vi "query Swept SA - Trace Value by CSV file.vi"(8 "error in (no error)":errorcluster, 10 "Trace Index":u32, 11 "Keysight 9020A in":refnum<class "Keysight 9020A.lvclass">) -> (0 "error out":errorcluster, 2 "Trace Values":T1 {"Frequency" format="%#_6p"}, 3 "Keysight 9020A out":refnum<class "Keysight 9020A.lvclass">)   [LabVIEW 2023, in "Spectrum Analyzer.lvlib" / "Keysight 9020A.lvclass"]
uses:
  Keysight 9020A.lvclass
  TYPE DEFINITION/TYPE Trace Value Array.ctl
  Keysight 9020A.lvclass/Keysight 9020A.ctl
  Spectrum Analyzer.lvlib
  <vilib>/Utility/file.llb/Read Delimited Spreadsheet (string).vi
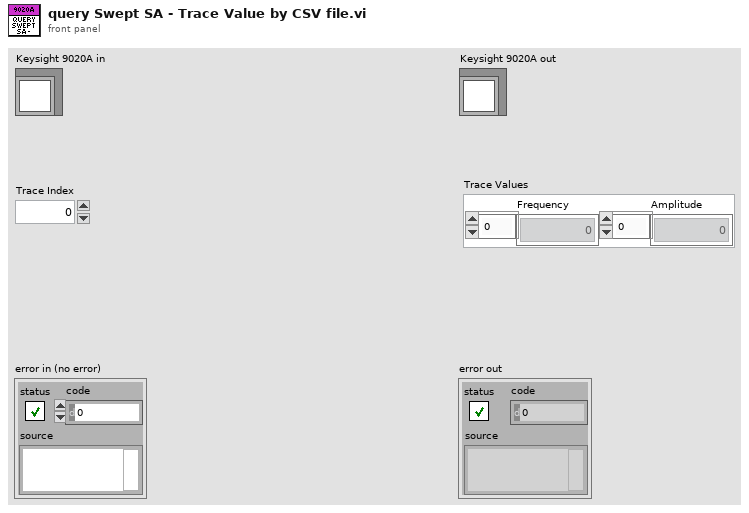
[diagram p1: front panel]
types:
  T1 = typedef "Spectrum Analyzer.lvlib/TYPE Trace Value Array.ctl" = cluster{"Frequency":dbl[], "Amplitude":dbl[]}
  T2 = enum16{"big-endian, network order", "native, host order", "little-endian"}
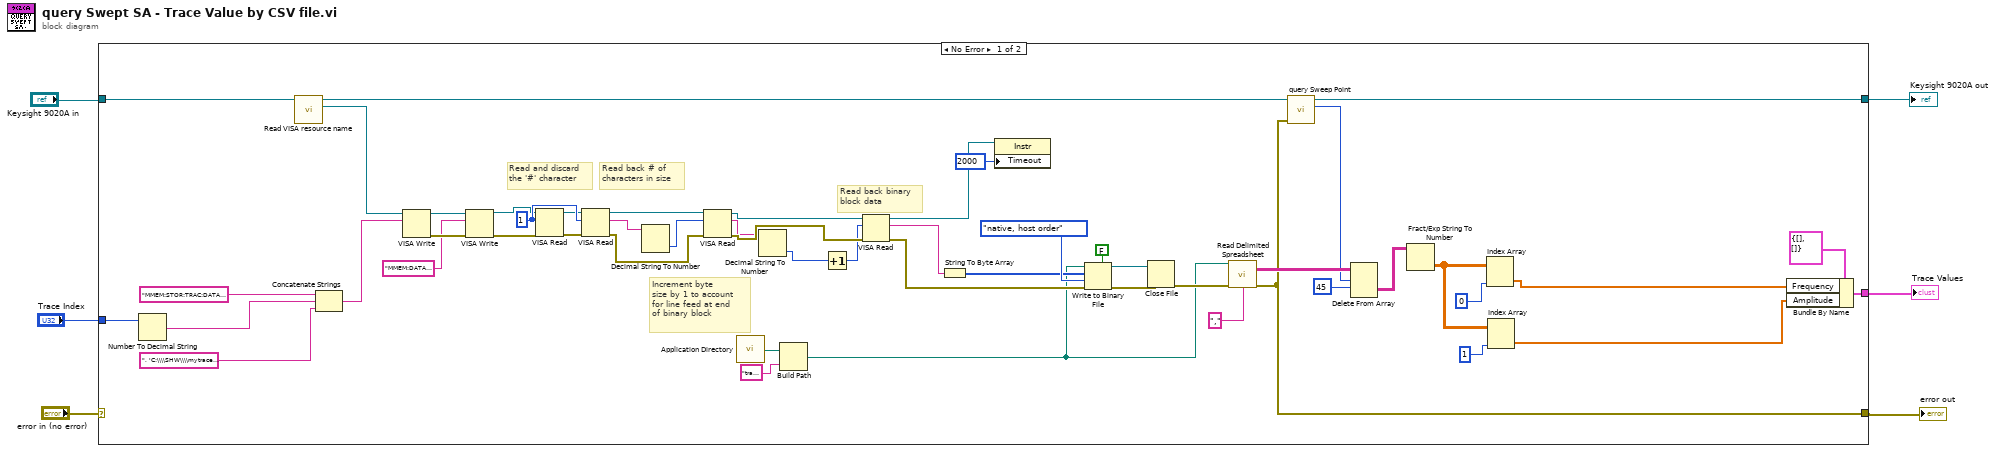
[diagram p0: block diagram]
diagram:
  n1 = case shown="No Error" "error in (no error)" {
    selector: "error in (no error)" -> [_ w59]
    tunnel: "Keysight 9020A in" -> [w58 w60]
    tunnel: [w15 w60] -> w5
    tunnel: [w14 w59] -> w2
    tunnel: "Trace Index" -> [w52 _]
    tunnel: [w56 _] -> w4
    frame No Error {
      w47 = u32 1 ("byte count")
      # "Read back binary\nblock data"
      # "Increment byte\nsize by 1 to account\nfor line feed at end\nof binary block"
      # "Read back # of\ncharacters in size"
      # "Read and discard\nthe '#' character"
      n2 = Number To Decimal String(number=w52) -> (decimal integer string=w54:string)  [unwired: 1 in]
      n3 = call "Read VISA resource name.vi"("Keysight 9020A in"=w58) -> ("VISA resource name"=w12:refnum<visa-resource-name>, "Keysight 9020A out"=w20:refnum<class "Keysight 9020A.lvclass">)  [unwired: 8 in, 1 out]
      n4 = Concatenate Strings("MMEM:STOR:TRAC:DATA TRACE" ("write buffer"), w54, ", 'C:\\\\SHW\\\\mytrace.csv';*OPC" ("write buffer")) -> (w51:string)
      n5 = VISA Write(VISA resource name=w12, write buffer=w51) -> (VISA resource name out=w50:refnum<visa-resource-name>, error out=w49:errorcluster)  [unwired: 1 in, 1 out]
      n6 = VISA Write(VISA resource name=w50, write buffer="MMEM:DATA? 'C:\\\\SHW\\\\mytrace.csv'", error in (no error)=w49) -> (VISA resource name out=w45:refnum<visa-resource-name>, error out=w44:errorcluster)  [unwired: 1 out]
      n7 = VISA Read(VISA resource name=w45, byte count=w47, error in (no error)=w44) -> (VISA resource name out=w46:refnum<visa-resource-name>, error out=w43:errorcluster)  [unwired: 2 out]
      n8 = VISA Read(VISA resource name=w46, byte count=w47, error in (no error)=w43) -> (VISA resource name out=w27:refnum<visa-resource-name>, read buffer=w25:string, error out=w26:errorcluster)  [unwired: 1 out]
      n9 = Decimal String To Number(string=w25) -> (number=w38:i32)  [unwired: 2 in, 1 out]
      n10 = VISA Read(VISA resource name=w27, byte count=w38, error in (no error)=w26) -> (VISA resource name out=w39:refnum<visa-resource-name>, read buffer=w40:string, error out=w42:errorcluster)  [unwired: 1 out]
      n11 = call <vilib>:"Application Directory.vi"() -> ("Application Directory"=w24:path)
      n12 = Decimal String To Number(string=w40) -> (number=w41:i32)  [unwired: 2 in, 1 out]
      n13 = Build Path(base path=w24, name or relative path="traceRawdata.csv") -> (appended path=w13:path)
      n14 = Increment(x=w41) -> (x+1=w31:i32)
      n15 = VISA Read(VISA resource name=w39, byte count=w31, error in (no error)=w42) -> (VISA resource name out=w28:refnum<visa-resource-name>, read buffer=w35:string, error out=w30:errorcluster)  [unwired: 1 out]
      n16 = String To Byte Array(string=w35) -> (unsigned byte array=w36:u8[])
      n17 = property class="Instr"(reference=w28, "Timeout"=u32 2000 ("General Settings:Timeout Value")) -> ()  [unwired: 1 in, 2 out]
      n18 = Write to Binary File(file (use dialog)=w13, data=w36, error in=w30, 5:FALSE ("prepend array or string size? (T)"), 9:T2."native, host order" ("byte order (0:big-endian, network order)")) -> (refnum out=w34:refnum<file>, error out=w33:errorcluster)  [unwired: 1 in, 1 out]
      n19 = Close File(refnum=w34, error in=w33) -> (error out=w21:errorcluster)  [unwired: 1 out]
      n20 = call-poly <vilib>:"Read Delimited Spreadsheet.vi"("file path (dialog if empty)"=w13, "error in (no error)"=w21, "delimiter (\\t)"="," ("delimiter (\\t)")) -> ("all rows"=w17:string[][], "error out"=w14:errorcluster)  [unwired: 7 in, 4 out]
      n21 = call-dynamic "query Sweep Point.vi"("error in (no error)"=w14, "Keysight 9020A in"=w20) -> ("Sweep Point"=w16:u32, "Keysight 9020A out"=w15:refnum<class "Keysight 9020A.lvclass">)  [unwired: 7 in, 1 out]
      n22 = Delete From Array(array=w17, length=w16, index (row)=45) -> (deleted portion=w18:string[][])  [unwired: 1 in, 1 out]
      n23 = Fract/Exp String To Number(string=w18) -> (number=w9:dbl[][])  [unwired: 3 in, 1 out]
      n24 = Index Array(array=w9, index (col)=0) -> (element=w10:dbl[])  [unwired: 1 in]
      n25 = Index Array(array=w9, index (col)=1) -> (element=w7:dbl[])  [unwired: 1 in]
      n26 = Bundle By Name(cluster=T1 {"Frequency"=[], "Amplitude"=[]} ("Trace Values 2"), "Frequency"=w10, "Amplitude"=w7) -> (w56:T1)
    }
    frame Error {
    }
  }
  "error out" <- w2
  "Keysight 9020A out" <- w5
  "Trace Values" <- w4
